vi "Get Frequency List - NF.vi"(11 "Measurement Configuration":T1={"Automation Test"=FALSE, "Power sequencing file path"="", "RFmx name"="5842", "RFmx port"="port1", "DUT Max Gain (dB)"=17.5, "DUT Max Noise Figure (dB)"=3.0, "Reference Level Mode"=enum."Recommend", "Reference Level (dBm)"=0.0, "Preamp Enabled"=3, "RFmx attenuation mode"=enum."<None>", "RFmx external attenuation (dB)"=0.8, "RFmx s-parameters orientation"=enum."Port1 Towards DUT", "RFmx s2p file path"="", "Switch Name"="2599_S8", "Switch Connection"="no0->com0", "ENS SMU Name"="", "ENS SMU Channel"="", "Action"=0, "Measurement Bandwidth (Hz)"=4000000.0, "Measurement Interval (s)"=0.1, "NF Cal Setup ID"="", "DUT Type"=0, "Frequency List Mode"=enum."Step", "Step - Start Frequency "=4000000000.0, "Step - Stop Frequency"=20000000000.0, "Step - Step Size"=1000000000.0, "Points - Start Frequency"=4000000000.0, "Points - Stop Frequency"=20000000000.0, "Points - Number of Points"=27, "FreqList - Frequency List"=[], "Averaging Enabled"=FALSE, "Averaging Count"=10, "Noise Source Type"=1, "Noise Source RFSG Port"="port2", "Noise Source Cold Temperature (K)"=302.8, "Noise Source Off Temperature (K)"=297.0, "ENR Freq (Hz)"=[6500000000.0], "ENR (dB)"=[15.0], "DUT Input_Compensation Enabled"=FALSE, "DUT Input_Temperation (K)"=297.0, "DUT Input_Loss Freq (Hz)"=[], "DUT Input_Loss (dB)"=[], "DUT Output_Compensation Enabled"=FALSE, "DUT Output_Temperation (K)"=297.0, "DUT Output_Loss Freq (Hz)"=[], "DUT Output_Loss (dB)"=[], "Calibration_Compensation Enabled"=FALSE, "Calibration_Temperation (K)"=297.0, "Calibration_Loss Freq (Hz)"=[], "Calibration_Loss (dB)"=[], "Noise Source_Compensation Enabled"=FALSE, "Noise Source_Temperation (K)"=297.0, "Noise Source_Loss Freq (Hz)"=[], "Noise Source_Loss (dB)"=[], "DUT Input Loss S2P File Path"="", "DUT Input Loss S-Parameter Orientation"=0, "DUT Output Loss S2P File Path"="", "DUT Output Loss S-Parameter Orientation"=0, "Calibration Loss S2P File Path"="", "Calibration Loss S-Parameter Orientation"=0, "Noise Source Loss S2P File Path"="", "Noise Source Loss S-Parameter Orientation"=0, "Power sequecing file validity check"=TRUE} {"Noise Source Loss S-Parameter Orientation" items=["Port1 Towards DUT", "Port2 Towards DUT"]; "Calibration Loss S-Parameter Orientation" items=["Port1 Towards DUT", "Port2 Towards DUT"]; "DUT Output Loss S-Parameter Orientation" items=["Port1 Towards DUT", "Port2 Towards DUT"]; "DUT Input Loss S-Parameter Orientation" items=["Port1 Towards DUT", "Port2 Towards DUT"]; "FreqList - Frequency List" format="%.3p Hz"; "Points - Stop Frequency" format="%.3p Hz"; "Points - Start Frequency" format="%.3p Hz"; "Step - Step Size" format="%.3p Hz"; "Step - Stop Frequency" format="%.3p Hz"; "Step - Start Frequency" format="%.3p Hz"; "Noise Source_Loss (dB)" format="%.2g"; "Noise Source_Loss Freq (Hz)" format="%.3p"; "Noise Source_Temperation (K)" format="%.2g"; "Calibration_Loss (dB)" format="%.2g"; "Calibration_Loss Freq (Hz)" format="%.3p"; "Calibration_Temperation (K)" format="%.2g"; "DUT Output_Loss (dB)" format="%.2g"; "DUT Output_Loss Freq (Hz)" format="%.3p"; "DUT Output_Temperation (K)" format="%.2g"; "DUT Input_Loss (dB)" format="%.2g"; "DUT Input_Loss Freq (Hz)" format="%.3p"; "DUT Input_Temperation (K)" format="%.2g"; "ENR (dB)" format="%.2g"; "ENR Freq (Hz)" format="%.3p"; "Noise Source Off Temperature (K)" format="%.2f"; "Noise Source Cold Temperature (K)" format="%.2f"; "Noise Source Type" items=["External Noise Source", "RF Signal Generator"]; "DUT Type" items=["Amplifier", "Downconverter", "Upconverter"]; "Measurement Interval (s)" format="%.2p"; "Measurement Bandwidth (Hz)" format="%.3p"; "Action" items=["Measure", "Calibrate"]; "RFmx external attenuation (dB)" format="%.2f"; "Preamp Enabled" items=["Disabled"=0, "Enabled"=1, "Automatic"=3]}) -> (3 "Frequency List":dbl[](array[numeric]) format="%.3p Hz")   [LabVIEW 2023, in "FPT NoiseFigure.lvclass"]
uses:
  FPT NoiseFigure.lvclass
  Measurement Configuration.ctl
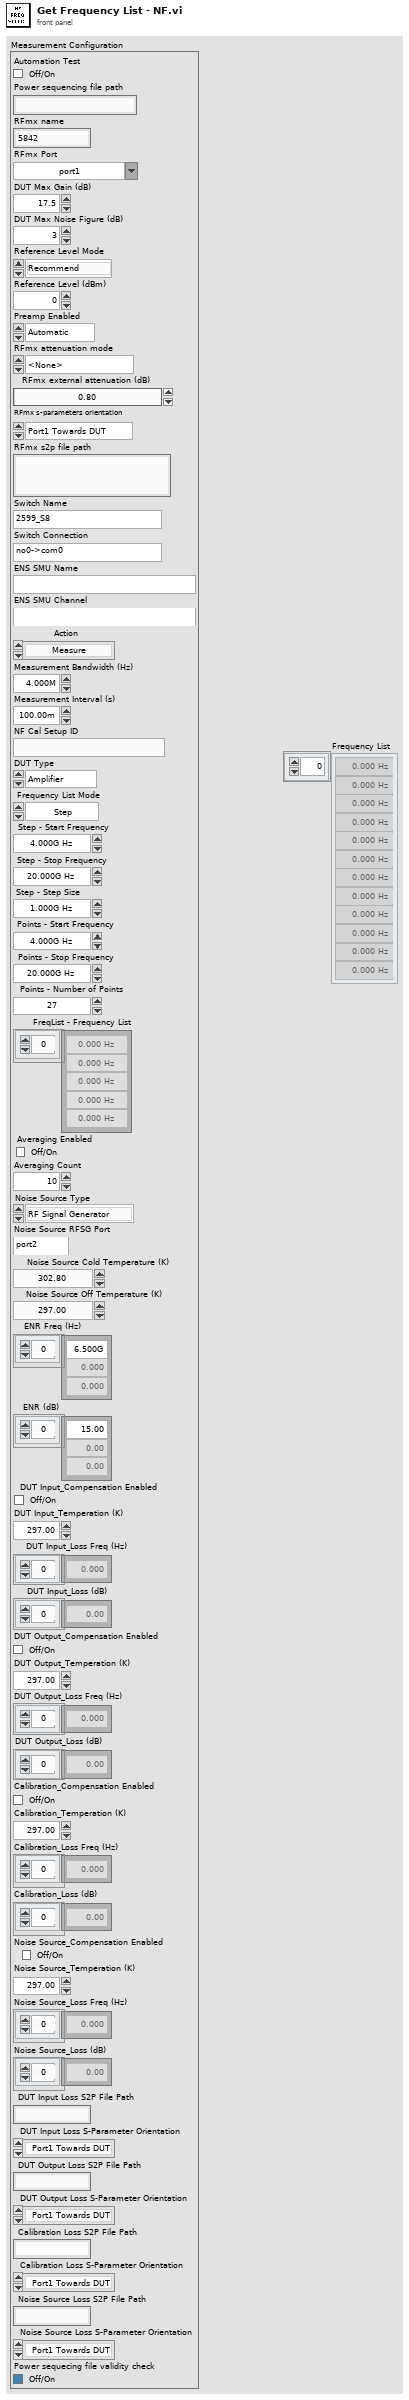
[diagram p1: front panel]
types:
  T1 = typedef "FPT NoiseFigure.lvclass/Measurement Configuration.ctl" = cluster{"Automation Test":bool, "Power sequencing file path":string, "RFmx name":string, "RFmx port":string, "DUT Max Gain (dB)":dbl, "DUT Max Noise Figure (dB)":dbl, "Reference Level Mode":enum32{"Manual", "Recommend"}, "Reference Level (dBm)":dbl, "Preamp Enabled":i32, "RFmx attenuation mode":enum32{"<None>", "Constant Attenuation", "s2p File"}, "RFmx external attenuation (dB)":dbl, "RFmx s-parameters orientation":enum32{"Port1 Towards DUT", "Port2 Towards DUT"}, "RFmx s2p file path":string, "Switch Name":string, "Switch Connection":string, "ENS SMU Name":string, "ENS SMU Channel":string, "Action":u32, "Measurement Bandwidth (Hz)":dbl, "Measurement Interval (s)":dbl, "NF Cal Setup ID":string, "DUT Type":i32, "Frequency List Mode":enum32{"Step", "Points", "Frequency List"}, "Step - Start Frequency ":dbl, "Step - Stop Frequency":dbl, "Step - Step Size":dbl, "Points - Start Frequency":dbl, "Points - Stop Frequency":dbl, "Points - Number of Points":i32, "FreqList - Frequency List":dbl[], "Averaging Enabled":bool, "Averaging Count":i32, "Noise Source Type":i32, "Noise Source RFSG Port":string, "Noise Source Cold Temperature (K)":dbl, "Noise Source Off Temperature (K)":dbl, "ENR Freq (Hz)":dbl[], "ENR (dB)":dbl[], "DUT Input_Compensation Enabled":bool, "DUT Input_Temperation (K)":dbl, "DUT Input_Loss Freq (Hz)":dbl[], "DUT Input_Loss (dB)":dbl[], "DUT Output_Compensation Enabled":bool, "DUT Output_Temperation (K)":dbl, "DUT Output_Loss Freq (Hz)":dbl[], "DUT Output_Loss (dB)":dbl[], "Calibration_Compensation Enabled":bool, "Calibration_Temperation (K)":dbl, "Calibration_Loss Freq (Hz)":dbl[], "Calibration_Loss (dB)":dbl[], "Noise Source_Compensation Enabled":bool, "Noise Source_Temperation (K)":dbl, "Noise Source_Loss Freq (Hz)":dbl[], "Noise Source_Loss (dB)":dbl[], "DUT Input Loss S2P File Path":string, "DUT Input Loss S-Parameter Orientation":i32, "DUT Output Loss S2P File Path":string, "DUT Output Loss S-Parameter Orientation":i32, "Calibration Loss S2P File Path":string, "Calibration Loss S-Parameter Orientation":i32, "Noise Source Loss S2P File Path":string, "Noise Source Loss S-Parameter Orientation":i32, "Power sequecing file validity check":bool}
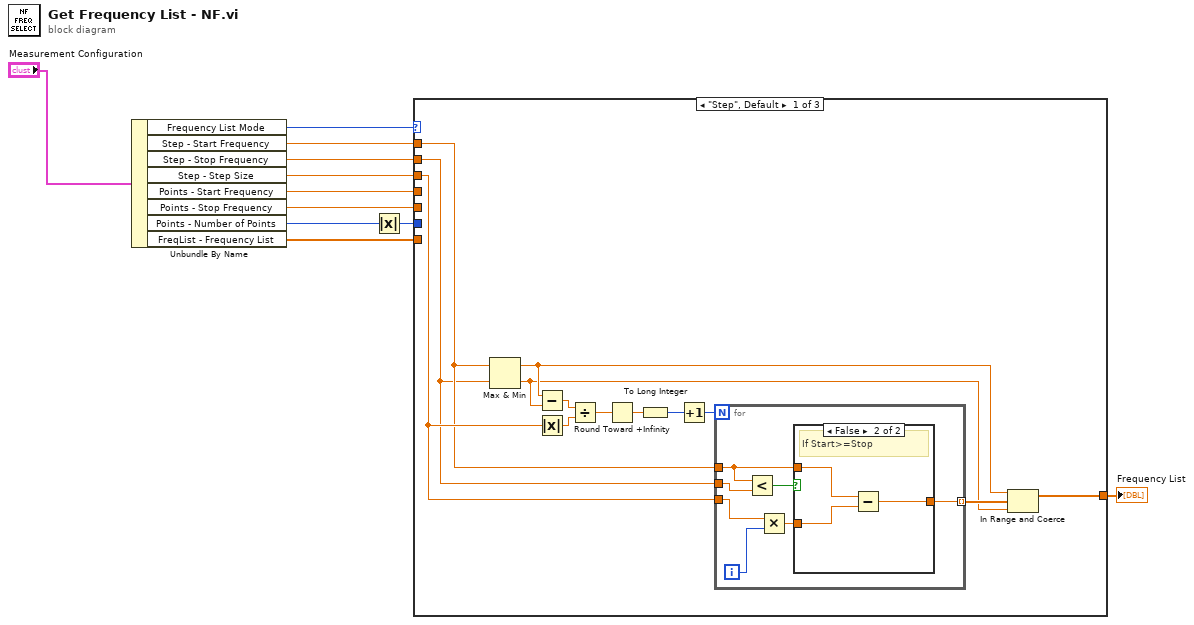
[diagram p0: block diagram]
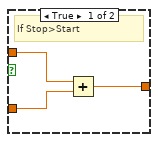
[diagram p2: hidden frame]
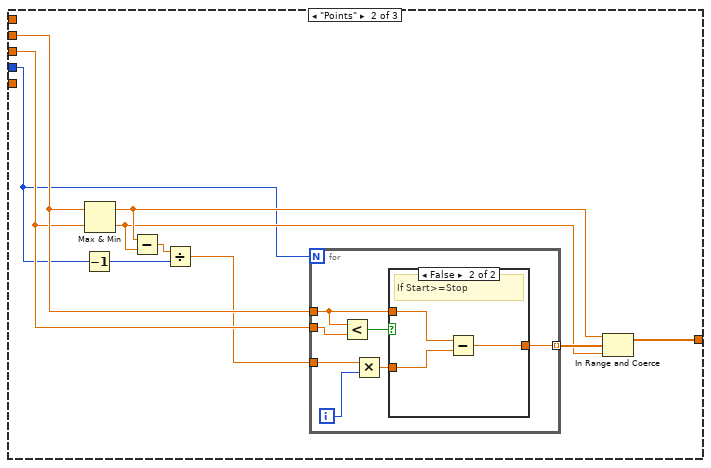
[diagram p3: hidden frame]
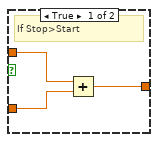
[diagram p4: hidden frame]
diagram:
  n1 = Unbundle By Name("Measurement Configuration") -> ("Frequency List Mode"=w2:enum32{"Step", "Points", "Frequency List"}, "Step - Start Frequency"=w11:dbl, "Step - Stop Frequency"=w10:dbl, "Step - Step Size"=w9:dbl, "Points - Start Frequency"=w7:dbl, "Points - Stop Frequency"=w6:dbl, "Points - Number of Points"=w5:i32, "FreqList - Frequency List"=w4:dbl[])
  n2 = Absolute Value(x=w5) -> (abs(x)=w3:i32)
  n3 = case shown="\"Step\", Default" w2 {
    tunnel: w11 -> [w19 _ _]
    tunnel: w10 -> [w18 _ _]
    tunnel: w9 -> [w21 _ _]
    tunnel: [w14 w43 w61] -> w8
    tunnel: w7 -> [_ w42 _]
    tunnel: w6 -> [_ w41 _]
    tunnel: w3 -> [_ w40 _]
    tunnel: w4 -> [_ _ w61]
    frame "Step", Default {
      n4 = Max & Min(x=w19, y=w18) -> (max(x,y)=w16:dbl, min(x,y)=w15:dbl)
      n5 = Subtract(x=w16, y=w15) -> (x-y=w17:dbl)
      n6 = Absolute Value(x=w21) -> (abs(x)=w24:dbl)
      n7 = Divide(x=w17, y=w24) -> (x/y=w23:dbl)
      n8 = Round Toward +Infinity(x=w23) -> (ceil(x): smallest int >= x=w12:dbl)
      n9 = To Long Integer(number=w12) -> (32bit integer=w22:i32)
      n10 = Increment(x=w22) -> (x+1=w13:i32)
      n11 = for {
        N: w13 -> [_]
        tunnel: w19 -> [w27]
        tunnel: w18 -> [w26]
        tunnel: w21 -> [w31]
        tunnel: [w25] -> w20 mode=indexing
        i -> [w30]
        n12 = Less?(x=w27, y=w26) -> (x < y?=w28:bool)
        n13 = Multiply(x=w31, y=w30) -> (x*y=w29:dbl)
        n14 = case shown="False" w28 {
          tunnel: w27 -> [w34 w37]
          tunnel: w29 -> [w33 w36]
          tunnel: [w32 w35] -> w25
          frame True {
            # "If Stop>Start"
            n15 = Add(x=w34, y=w33) -> (x+y=w32:dbl)
          }
          frame False {
            # "If Start>=Stop"
            n16 = Subtract(x=w37, y=w36) -> (x-y=w35:dbl)
          }
        }
      }
      n17 = In Range and Coerce(upper limit=w16, x=w20, lower limit=w15) -> (coerced(x)=w14:dbl[])  [unwired: 1 out]
    }
    frame "Points" {
      n18 = Decrement(x=w40) -> (x-1=w38:i32)
      n19 = Max & Min(x=w42, y=w41) -> (max(x,y)=w45:dbl, min(x,y)=w44:dbl)
      n20 = Subtract(x=w45, y=w44) -> (x-y=w46:dbl)
      n21 = Divide(x=w46, y=w38) -> (x/y=w39:dbl)
      n22 = for {
        N: w40 -> [_]
        tunnel: w42 -> [w51]
        tunnel: w41 -> [w50]
        tunnel: [w49] -> w47 mode=indexing
        tunnel: w39 -> [w48]
        i -> [w54]
        n23 = Less?(x=w51, y=w50) -> (x < y?=w52:bool)
        n24 = Multiply(x=w48, y=w54) -> (x*y=w53:dbl)
        n25 = case shown="False" w52 {
          tunnel: w51 -> [w57 w60]
          tunnel: w53 -> [w56 w59]
          tunnel: [w55 w58] -> w49
          frame True {
            # "If Stop>Start"
            n26 = Add(x=w57, y=w56) -> (x+y=w55:dbl)
          }
          frame False {
            # "If Start>=Stop"
            n27 = Subtract(x=w60, y=w59) -> (x-y=w58:dbl)
          }
        }
      }
      n28 = In Range and Coerce(upper limit=w45, x=w47, lower limit=w44) -> (coerced(x)=w43:dbl[])  [unwired: 1 out]
    }
    frame "Frequency List" {
    }
  }
  "Frequency List" <- w8
